vi "UMLEditor ToolsMenuUpdates.vi"(0 "menu":refnum<k9>, 2 "item":string, 3 "Graph":refnum<class "Graph.lvclass">, 5 "error in (no error)":errorcluster) -> (19 "error out":errorcluster)   [LabVIEW 2020]
doc: "Gets current diagram values"
uses:
  <resource>/Framework/Providers/Open_GDS/UML/Graph_class/Graph.lvclass
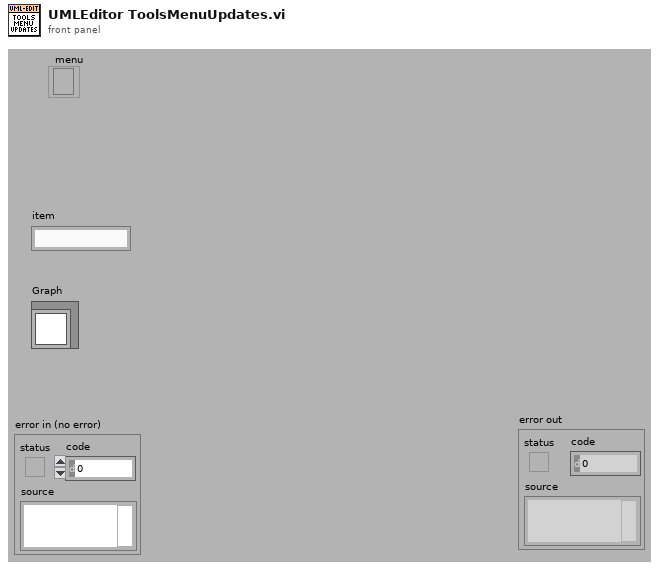
[diagram p1: front panel]
types:
  T1 = cluster{string, string, "short cut out":cluster{"include Shift key?":bool, "include Ctrl key? ":bool, "shortcut key":string}}[]
  T2 = cluster{"include Shift key?":bool, "include Ctrl key? ":bool, "shortcut key":string}
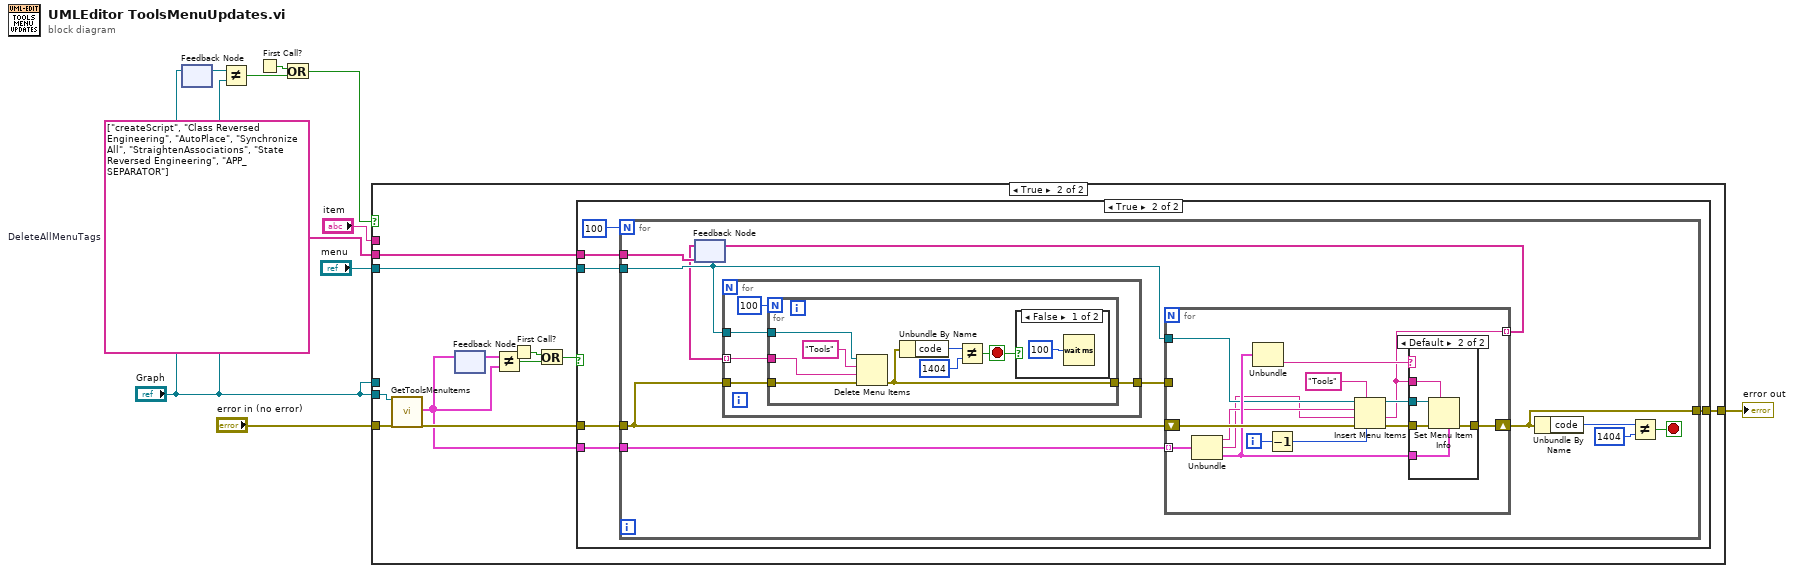
[diagram p0: block diagram]
diagram:
  w6 = string[] ["createScript", "Class Reversed Engineering", "AutoPlace", "Synchronize All", "StraightenAssociations", "State Reversed Engineering", "APP_SEPARATOR"]  # DeleteAllMenuTags
  n1 = feedback #1() -> (w5:refnum<class "Graph.lvclass">)  [unwired: 1 in]
  n2 = feedback-in #1("Graph") -> ()
  n3 = Not Equal?(x=w5, y="Graph") -> (x != y?=w3:bool)
  n4 = First Call?() -> (First Call?: T/F=w4:bool)
  n5 = Or(x=w4, y=w3) -> (x .or. y?=w2:bool)
  n6 = case shown="True" w2 {
    tunnel: [w11 w22] -> w9
    tunnel: "menu" -> [_ w21]
    tunnel: "Graph" -> [_ _]
    tunnel: "item" -> [_ _]
    tunnel: "error in (no error)" -> [w11 w20]
    tunnel: w6 -> [_ w18]
    tunnel: "Graph" -> [_ w19]
    frame False {
    }
    frame True {
      n7 = call-dynamic "GetToolsMenuItems.vi"("reference in"=w19, "error in (no error)"=w20) -> ("ToolMenuItems"=w13:T1, "error out"=w17:errorcluster)  [unwired: 15 in, 1 out]
      n8 = feedback #2() -> (w14:T1)  [unwired: 1 in]
      n9 = feedback-in #2(w13) -> ()
      n10 = Not Equal?(x=w14, y=w13) -> (x != y?=w16:bool)
      n11 = First Call?() -> (First Call?: T/F=w15:bool)
      n12 = Or(x=w15, y=w16) -> (x .or. y?=w12:bool)
      n13 = case shown="True" w12 {
        tunnel: [w23 w29] -> w22
        tunnel: w21 -> [_ w28]
        tunnel: w18 -> [_ w27]
        tunnel: w17 -> [w23 w26]
        tunnel: w13 -> [_ w24]
        frame False {
        }
        frame True {
          n14 = for {
            N: 100 -> [_]
            tunnel: w28 -> [w40]
            tunnel: w24 -> [w39]
            tunnel: w27 -> [w37]
            tunnel: w26 -> [w34]
            tunnel: [w31] -> w29
            stop <- w30 stop-if-true
            n15 = feedback #3(w37) -> (w36:string[])
            n16 = for {
              tunnel: w40 -> [w45]
              tunnel: w36 -> [w44] mode=indexing
              tunnel: w34 -> [w41]
              tunnel: [w43] -> w35
              n17 = for {
                N: 100 -> [_]
                tunnel: w45 -> [w53]
                tunnel: w44 -> [w50]
                tunnel: w41 -> [w51]
                tunnel: [w49] -> w43
                stop <- w46 stop-if-true
                n18 = Delete Menu Items(6:w51, 7:w50, 8:"Tools" ("item tag"), 9:w53) -> (0:w49:errorcluster)  [unwired: 1 out]
                n19 = Unbundle By Name(w49) -> ("code"=w48:i32)
                n20 = Not Equal?(x=w48, y=1404) -> (x != y?=w46:bool)
                n21 = case shown="False" w46 {
                  frame False {
                    n22 = Wait (ms)(milliseconds to wait=u32 100) -> ()  [unwired: 1 out]
                  }
                  frame True {
                  }
                }
              }
            }
            n23 = for {
              tunnel: w39 -> [w66] mode=indexing
              shift-right: [w61] -> w31
              shift-left: w34 -> [w65]
              tunnel: w40 -> [w62]
              tunnel: [w55] -> w38 mode=indexing
              tunnel: w35 -> [_]
              i -> [w59]
              n24 = Unbundle(w66) -> (w63:string, w56:string, "short cut out"=w64:T2)
              n25 = Unbundle(w64) -> ("shortcut key"=w57:string)  [unwired: 2 out]
              n26 = Decrement(x=w59) -> (x-1=w58:i32)
              n27 = Insert Menu Items(4:w58, 5:"Tools" ("menu tag"), 6:w65, 7:w56, 8:w63, 9:w62) -> (0:w60:errorcluster, 1:w55:string, 3:w67:refnum<k9>)
              n28 = case shown="Default" w57 {
                tunnel: w67 -> [_ w74]
                tunnel: w64 -> [_ w70]
                tunnel: w55 -> [_ w73]
                tunnel: [w69 w72] -> w61
                tunnel: w60 -> [w69 w71]
                frame "" {
                }
                frame Default {
                  n29 = Set Menu Item Info(4:w70, 7:w73, 8:w71, 11:w74) -> (0:w72:errorcluster)  [unwired: 4 out]
                }
              }
            }
            n30 = feedback-in #3(w38) -> ()
            n31 = Unbundle By Name(w31) -> ("code"=w32:i32)
            n32 = Not Equal?(x=w32, y=1404) -> (x != y?=w30:bool)
          }
        }
      }
    }
  }
  "error out" <- w9
